vi "Post-Install Custom Action.vi"(10 "Variant":variant) -> (0 "error out":errorcluster)   [LabVIEW 2020]
uses:
  <vilib>/Utility/traverseref.llb/TRef TravTarget.ctl
  <vilib>/Utility/traverseref.llb/VI Scripting - Traverse.lvlib
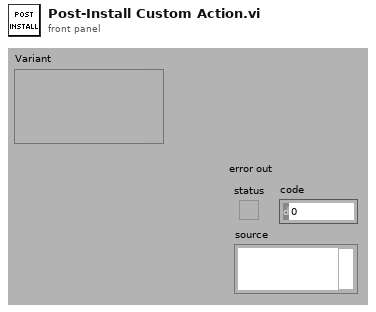
[diagram p1: front panel]
types:
  T1 = typedef "TRef TravTarget.ctl" = enum16{"FP", "BD", "Other"}
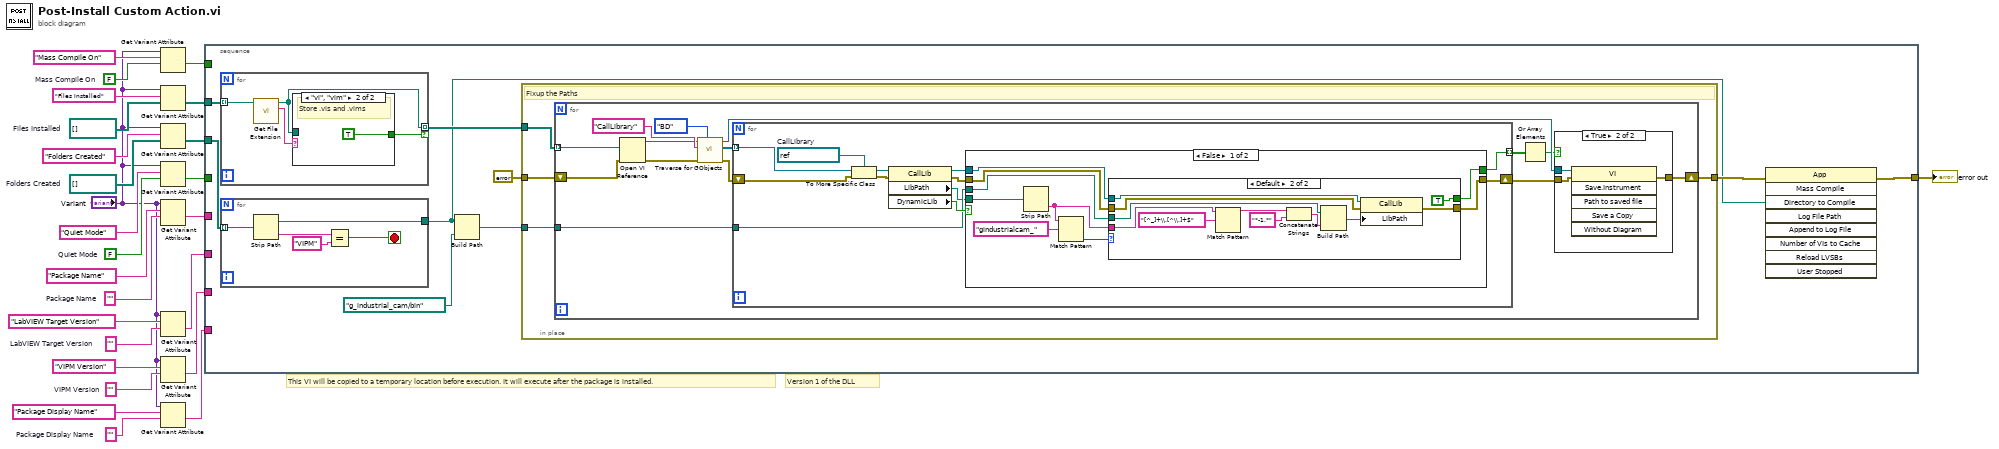
[diagram p0: block diagram]
diagram:
  w3 = path[] []  # Folders Created
  w4 = path[] []  # Files Installed
  w9 = FALSE  # Mass Compile On
  w10 = ""  # Package Display Name
  w17 = FALSE  # Quiet Mode
  w20 = ""  # VIPM Version
  w22 = ""  # LabVIEW Target Version
  w24 = ""  # Package Name
  # "Version 1 of the DLL"
  # "This VI will be copied to a temporary location before execution. It will execute after the package is installed."
  n1 = Get Variant Attribute(Variant="Variant", name="Mass Compile On", default value (empty Variant)=w9) -> (value=w11:bool)  [unwired: 1 in, 3 out]
  n2 = Get Variant Attribute(Variant="Variant", name="Files Installed", default value (empty Variant)=w4) -> (value=w6:path[])  [unwired: 1 in, 3 out]
  n3 = Get Variant Attribute(Variant="Variant", name="Folders Created", default value (empty Variant)=w3) -> (value=w7:path[])  [unwired: 1 in, 3 out]
  n4 = Get Variant Attribute(Variant="Variant", name="Quiet Mode", default value (empty Variant)=w17) -> (value=w12:bool)  [unwired: 1 in, 3 out]
  n5 = Get Variant Attribute(Variant="Variant", name="Package Name", default value (empty Variant)=w24) -> (value=w15:string)  [unwired: 1 in, 3 out]
  n6 = Get Variant Attribute(Variant="Variant", name="LabVIEW Target Version", default value (empty Variant)=w22) -> (value=w14:string)  [unwired: 1 in, 3 out]
  n7 = Get Variant Attribute(Variant="Variant", name="VIPM Version", default value (empty Variant)=w20) -> (value=w13:string)  [unwired: 1 in, 3 out]
  n8 = Get Variant Attribute(Variant="Variant", name="Package Display Name", default value (empty Variant)=w10) -> (value=w16:string)  [unwired: 1 in, 3 out]
  n9 = stacked-sequence {
    tunnel: w16 -> [_]
    tunnel: w15 -> [_]
    tunnel: w14 -> [_]
    tunnel: w13 -> [_]
    tunnel: w12 -> [_]
    tunnel: w11 -> [_]
    tunnel: w6 -> [w35]
    tunnel: w7 -> [w34]
    tunnel: [w28] -> w2
    frame #0 {
      n10 = for {
        tunnel: w35 -> [w44] mode=indexing
        tunnel: [w41] -> w33 mode=indexing if=w42
        n11 = call <vilib>:"Get File Extension.vi"("file"=w44) -> ("lowercase file extension"=w43:string, "dup file"=w41:path)  [unwired: 6 in, 3 out]
        n12 = case shown="\"vi\", \"vim\"" w43 {
          tunnel: [_ TRUE] -> w42
          tunnel: w41 -> [_ _]
          frame Default {
          }
          frame "vi", "vim" {
            # "Store .vis and .vims"
          }
        }
      }
      n13 = for {
        tunnel: w34 -> [w40] mode=indexing
        tunnel: [w39] -> w27
        stop <- w37 stop-if-true
        n14 = Strip Path(path=w40) -> (stripped path=w39:path, name=w38:string)
        n15 = Equal?(x=w38, y="VIPM") -> (x = y?=w37:bool)
      }
      n16 = Build Path(base path=w27, name or relative path=path "g_industrial_cam/bin") -> (appended path=w31:path)
      n17 = in-place {
        in-place-border: [w47] -> w30
        in-place-border: w33 -> [w49]
        in-place-border: errorcluster {"status"=FALSE, "code"=0, "source"=""} ("error in (no error)") -> [w48]
        in-place-border: w31 -> [w46]
        # "Fixup the Paths"
        n18 = for {
          tunnel: w49 -> [w61] mode=indexing
          shift-right: [w59] -> w47
          shift-left: w48 -> [w58]
          tunnel: w46 -> [w50]
          n19 = Open VI Reference(vi path=w61, error in (no error)=w58) -> (vi reference=w54:refnum<vi>, error out=w53:errorcluster)  [unwired: 4 in]
          n20 = call <vilib>:"Traverse for GObjects.vi"("Traverse Target"=TRef_TravTarget."BD", "error in (no error)"=w53, "Class Name"="CallLibrary", "VI Refnum"=w54) -> ("error out"=w57:errorcluster, "References"=w52:refnum<vi>[], "dup VI Refnum"=w63:refnum<vi>)  [unwired: 4 in, 1 out]
          n21 = for {
            tunnel: w52 -> [w68] mode=indexing
            shift-right: [w75] -> w62
            shift-left: w57 -> [w70]
            tunnel: [w66] -> w51 mode=indexing
            tunnel: w50 -> [w65]
            w69 = refnum<vi> refnum  # CallLibrary
            n22 = To More Specific Class(target class=w69, reference=w68, error in=w70) -> (specific class reference=w71:refnum<vi>, error out=w72:errorcluster)
            n23 = property class="CallLib"(reference=w71, error in=w72) -> (reference out=w74:refnum<vi>, error out=w73:errorcluster, "LibPath"=w64:path, "DynamicLib"=w67:bool)
            n24 = case shown="False" w67 {
              tunnel: [w84 w97] -> w75
              tunnel: w74 -> [w83 _]
              tunnel: w73 -> [w82 w97]
              tunnel: w64 -> [w80 _]
              tunnel: [w79 _] -> w66
              tunnel: w65 -> [w77 _]
              frame False {
                n25 = Strip Path(path=w80) -> (name=w76:string)  [unwired: 1 out]
                n26 = Match Pattern(string=w76, regular expression="gindustrialcam_") -> (offset past match=w78:i32)  [unwired: 1 in, 3 out]
                n27 = case shown="Default" w78 {
                  tunnel: [w85 w96] -> w84
                  tunnel: w83 -> [_ w94]
                  tunnel: w82 -> [w85 w93]
                  tunnel: [_ TRUE] -> w79
                  tunnel: w77 -> [_ w91]
                  tunnel: w76 -> [_ w87]
                  frame -1 {
                  }
                  frame Default {
                    n28 = Match Pattern(string=w87, regular expression="[^_]+\\.[^\\.]+$") -> (before substring=w90:string)  [unwired: 1 in, 3 out]
                    n29 = Concatenate Strings(w90, "*-1.*" ("string")) -> (w86:string)
                    n30 = Build Path(base path=w91, name or relative path=w86) -> (appended path=w95:path)
                    n31 = property class="CallLib"(reference=w94, error in=w93, "LibPath"=w95) -> (error out=w96:errorcluster)  [unwired: 1 out]
                  }
                }
              }
              frame True {
              }
            }
          }
          n32 = Or Array Elements(Boolean array=w51) -> (logical OR=w60:bool)
          n33 = case shown="True" w60 {
            tunnel: w63 -> [_ w100]
            tunnel: w62 -> [w98 w99]
            tunnel: [w98 w101] -> w59
            frame False {
            }
            frame True {
              n34 = invoke class="VI" method="Save.Instrument"(reference=w100, error in=w99) -> (error out=w101:errorcluster)  [unwired: 4 in, 5 out]
            }
          }
        }
      }
      n35 = invoke class="App" method="Mass Compile"(error in=w30, "Directory to Compile"=w27) -> (error out=w28:errorcluster)  [unwired: 7 in, 8 out]
    }
  }
  "error out" <- w2
